vi "Image_Load.vi"(0 "File name":string="hud.png", 11 "error in":errorcluster) -> (4 "Image":T1, 15 "error out":errorcluster)   [LabVIEW 2020, in "GH_Render.lvlib"]
doc: "Loads a PNG from Resources\\Images as image data (24 bit, no transparency), e.g. a room background or the HUD."
uses:
  GH_Render.lvlib
  Level/GH_Level.lvlib
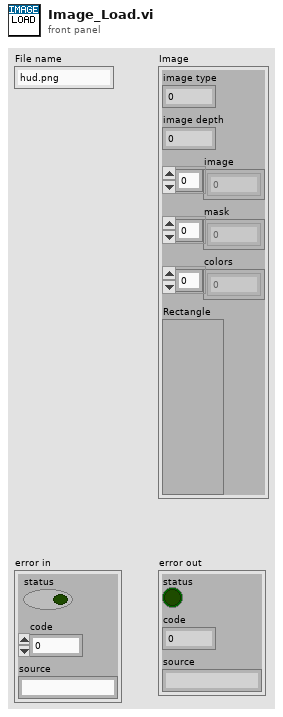
[diagram p1: front panel]
types:
  T1 = cluster{"image type":i32, "image depth":i32, "image":u8[], "mask":u8[], "colors":u32[], "Rectangle":cluster{"left":i16, "top":i16, "right":i16, "bottom":i16}}
  T2 = typedef "imagedata.ctl" = cluster{"image type":i32, "image depth":i32, "image":u8[], "mask":u8[], "colors":u32[], "Rectangle":cluster{"left":i16, "top":i16, "right":i16, "bottom":i16}}
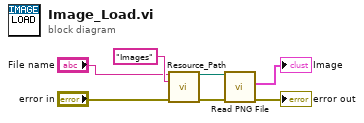
[diagram p0: block diagram]
diagram:
  n1 = call "Resource_Path.vi"("File name"="File name", "Subfolder"="Images", "error in"="error in") -> ("Path"=w4:path, "error out"=w5:errorcluster)  [unwired: 11 in]
  n2 = call <vilib>:"Read PNG File.vi"("error in (no error)"=w5, "path to PNG file"=w4) -> ("error out"=→"error out":errorcluster, "image data"=→"Image":T2)  [unwired: 7 in, 1 out]
